vi "SPARK Get Device Status.vi"   [LabVIEW 2023]
doc: "Get the status of the SPARK."
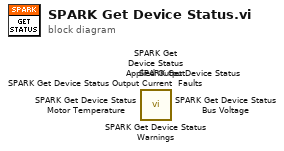
[diagram p0: block diagram]
diagram:
  n1 = call <vilib>:"SPARK Get Device Status Warnings.vi"() -> ()  [unwired: 7 in, 5 out]
  n2 = call <vilib>:"SPARK Get Device Status Faults.vi"() -> ()  [unwired: 7 in, 5 out]
  n3 = call <vilib>:"SPARK Get Device Status Motor Temperature.vi"() -> ()  [unwired: 8 in, 4 out]
  n4 = call <vilib>:"SPARK Get Device Status Bus Voltage.vi"() -> ()  [unwired: 8 in, 4 out]
  n5 = call <vilib>:"SPARK Get Device Status Output Current.vi"() -> ()  [unwired: 8 in, 4 out]
  n6 = call <vilib>:"SPARK Get Device Status Applied Output.vi"() -> ()  [unwired: 8 in, 4 out]
